vi "Remote Client Metrics.vi"() -> ()   [LabVIEW 2019]
uses:
  lvsrc/SMOs/RemoteControl/Typedefs/RC Com Type--enum.ctl
  lvsrc/SMOs/RemoteControl/RemoteControl.lvclass
panel:
  in  "RC Type":T1
  in  "stop":bool
  out "time":cluster{i32[], i32[]}[](graph)
  in  "Number of Messages":i32=20
  in  "step":dbl
  in  "end":dbl
  in  "start":dbl
  out "throughput":cluster{i32[], dbl[]}[](graph)
  out "message rate":cluster{i32[], dbl[]}[](graph)
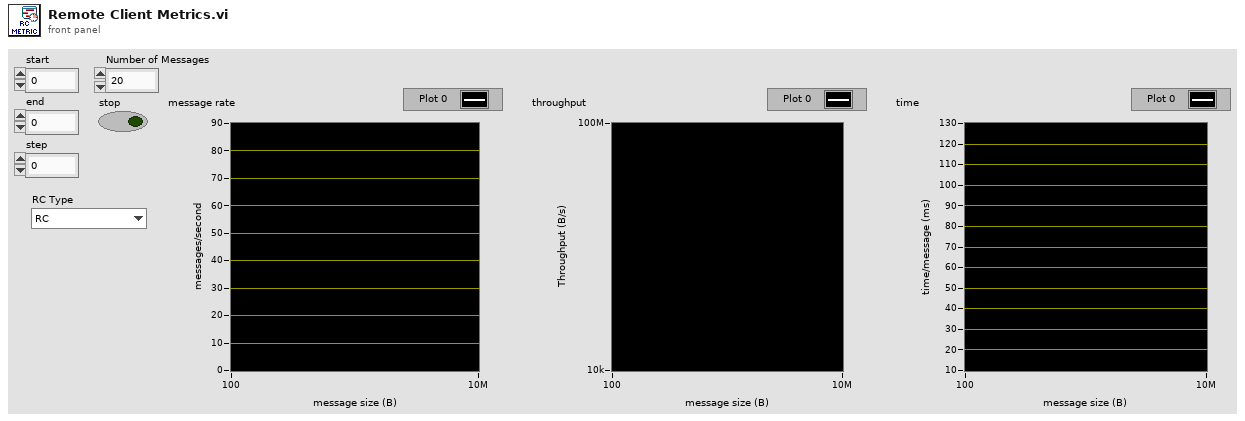
[diagram p1: front panel]
types:
  T1 = typedef "RemoteControl.lvclass/RC Com Type--enum.ctl" = enum16{"RC", "STM", "ZMQ"}
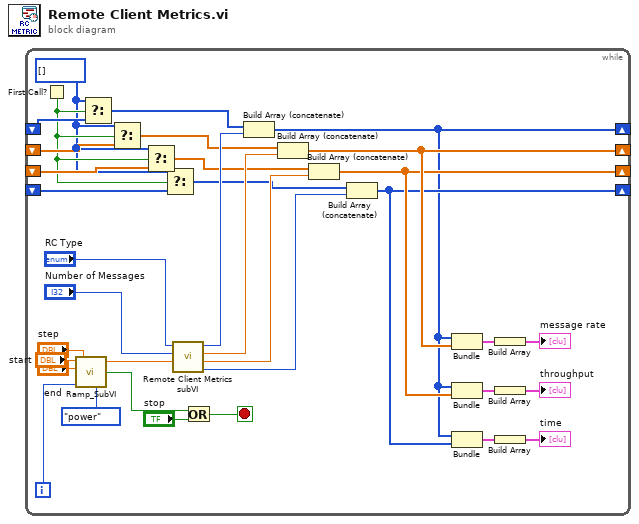
[diagram p0: block diagram]
diagram:
  n1 = while {
    shift-right: [w11] -> _
    shift-left: _ -> [w25]
    shift-right: [w17] -> _
    shift-left: _ -> [w23]
    shift-right: [w16] -> _
    shift-left: _ -> [w24]
    shift-right: [w15] -> _
    shift-left: _ -> [w12]
    i -> [w33]
    stop <- w3 stop-if-true
    w4 = i32[] [] ("t")
    n2 = First Call?() -> (First Call?: T/F=w18:bool)
    n3 = call <userlib>:"Ramp_SubVI.vi"("Enum"=enum16{"linear", "power"}."power", "index"=w33, "step"="step", "end"="end", "start"="start") -> ("Stop?"=w34:bool, "Numeric"=w14:dbl)
    n4 = Select(t=w4, s=w18, f=w25) -> (s? t:f=w22:i32[])
    n5 = Select(t=w4, s=w18, f=w23) -> (s? t:f=w21:dbl[])
    n6 = Select(t=w4, s=w18, f=w24) -> (s? t:f=w20:dbl[])
    n7 = Select(t=w4, s=w18, f=w12) -> (s? t:f=w19:i32[])
    n8 = call "Remote Client Metrics subVI.vi"("Message size"=w14, "Number of Messages"="Number of Messages", "RC Type"="RC Type") -> ("<time/message (ms)>"=w26:i32, "bytes/second"=w27:dbl, "messages/second"=w28:dbl, "<size>"=w29:i32)  [unwired: 5 in]
    n9 = Or(x=w34, y="stop") -> (x .or. y?=w3:bool)
    n10 = Build Array (concatenate)(w22, w29) -> (w11:i32[])
    n11 = Build Array (concatenate)(w21, w28) -> (w17:dbl[])
    n12 = Build Array (concatenate)(w20, w27) -> (w16:dbl[])
    n13 = Build Array (concatenate)(w19, w26) -> (w15:i32[])
    n14 = Bundle(w11, w17) -> (w10:cluster{i32[], dbl[]})  [unwired: 1 in]
    n15 = Bundle(w11, w16) -> (w8:cluster{i32[], dbl[]})  [unwired: 1 in]
    n16 = Bundle(w11, w15) -> (w7:cluster{i32[], i32[]})  [unwired: 1 in]
    n17 = Build Array(w10) -> (→"message rate":cluster{i32[], dbl[]}[])
    n18 = Build Array(w8) -> (→"throughput":cluster{i32[], dbl[]}[])
    n19 = Build Array(w7) -> (→"time":cluster{i32[], i32[]}[])
  }
